vi "Assert Not Error.vi"(4 "Execution time (s)":dbl=-1.0, 5 "Assert Only? (F)":bool, 6 "error code (1)":i32=1, 7 "Label":string, 8 "error in (no error)":errorcluster, 9 "Register with caller test (F)":bool, 11 "Not Error?":errorcluster) -> (0 "error out":errorcluster, 2 "Properties.Assert":refnum<class "Properties.Assert.lvclass">)   [LabVIEW 2020, in "Caraya.lvlib" / "Assert.lvclass"]
doc: "Generates an error if the input condition is not met.\n\n--\nCopyright © 2015 JKI All rights reserved.\n\nAuthor: Tomi Maila <tomi.maila@jki.net>\n\nThis library is provided \"AS IS\" ,WITHOUT WARRANTIES OR\nCONDITIONS OF ANY KIND, either express or implied.\n\nJKI -- jki.net"
uses:
  Assert.lvclass
  Properties.Assert/Properties.Assert.lvclass
  C:/projects/caraya/src/classes/Properties/Properties.lvclass
  Properties/Properties.lvclass
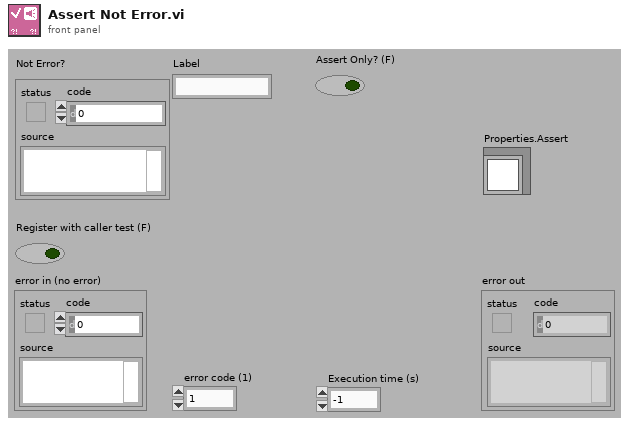
[diagram p1: front panel]
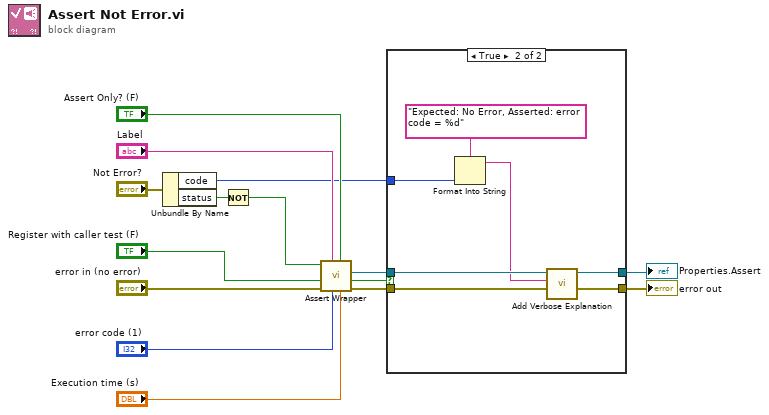
[diagram p0: block diagram]
diagram:
  n1 = Unbundle By Name("Not Error?") -> ("code"=w5:i32, "status"=w12:bool)
  n2 = Not(x=w12) -> (.not. x?=w11:bool)
  n3 = call "Assert Wrapper.vi"("Execution time (s)"="Execution time (s)", "Assert Only? (F)"="Assert Only? (F)", "error code (1)"="error code (1)", "Label"="Label", "error in (no error)"="error in (no error)", "Register with caller test (F)"="Register with caller test (F)", "Assert?"=w11) -> ("error out"=w8:errorcluster, "Verbose"=w4:bool, "Properties.Assert"=w2:refnum<class "Properties.Assert.lvclass">)  [unwired: 1 in, 1 out]
  n4 = case shown="True" w4 {
    tunnel: [w17 w19] -> w6
    tunnel: w8 -> [w17 w21]
    tunnel: w5 -> [_ w23]
    tunnel: w2 -> [w16 w22]
    tunnel: [w16 w18] -> w1
    frame False {
    }
    frame True {
      n5 = Format Into String(format string="Expected: No Error, Asserted: error code = %d", w23) -> (resulting string=w20:string)  [unwired: 2 in, 1 out]
      n6 = call "Add Verbose Explanation.vi"("error in (no error)"=w21, "Verbose Explanation"=w20, "Properties"=w22) -> ("error out"=w19:errorcluster, "Properties"=w18:refnum<class "Properties.Assert.lvclass">)  [unwired: 7 in]
    }
  }
  "error out" <- w6
  "Properties.Assert" <- w1
